vi "ReadConfigurationFile.vi"(8 "error in (no error)":errorcluster, 11 "object in":refnum<class "Configuration.lvclass">) -> (0 "error out":errorcluster, 2 "Configuration File":path, 3 "object out":refnum<class "Configuration.lvclass">)   [LabVIEW 2021, in "Channel.lvlib" / "Configuration.lvclass"]
uses:
  Configuration.lvclass
  Configuration.lvclass/Configuration.ctl
  Channel.lvlib
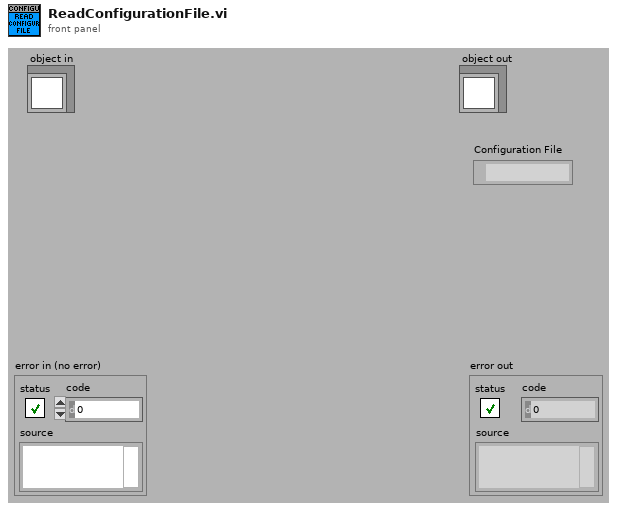
[diagram p1: front panel]
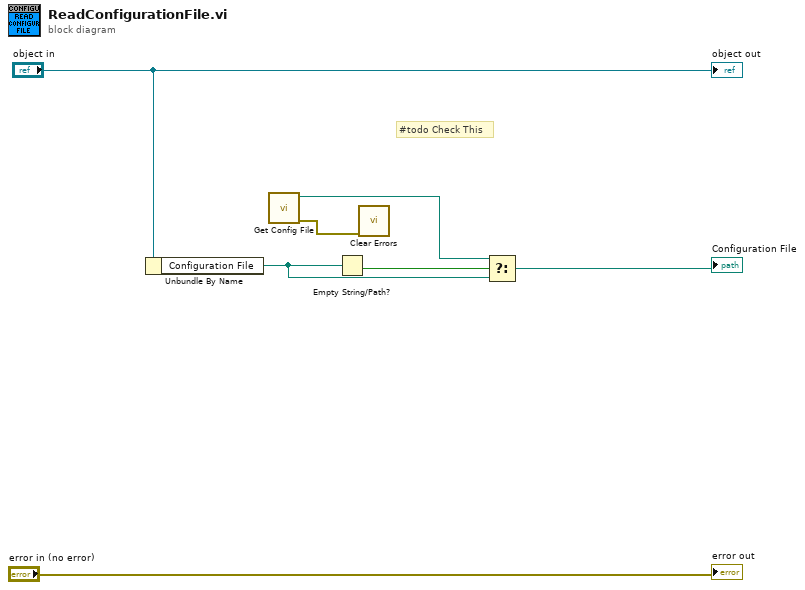
[diagram p0: block diagram]
diagram:
  # "#todo Check This"
  n1 = Unbundle By Name("object in") -> ("Configuration File"=w3:path)
  n2 = call "Get Config File.vi"() -> ("error out"=w1:errorcluster, "Config File"=w4:path)  [unwired: 10 in]
  n3 = Empty String/Path?(string/path=w3) -> (empty?=w5:bool)
  n4 = call <vilib>:"Clear Errors.vi"("error in (no error)"=w1) -> ()  [unwired: 5 in, 2 out]
  n5 = Select(t=w4, s=w5, f=w3) -> (s? t:f=→"Configuration File":path)
  "error out" <- "error in (no error)"
  "object out" <- "object in"
